vi "Set Setpoints.vi"(8 "error in":errorcluster, 10 "Plant Setpoints":T1, 11 "Sim Plant in":refnum<class "Sim Plant.lvclass">) -> (0 "error out":errorcluster, 3 "Sim Plant out":refnum<class "Sim Plant.lvclass">)   [LabVIEW 2026, in "Sim Plant.lvclass"]
doc: "Stores new plant setpoints. The plant model moves towards them on every Tick. Message: Set Setpoints Msg (payload Plant Setpoints)."
uses:
  Sim Plant.lvclass
  Sim Plant.lvclass/Sim Plant.ctl
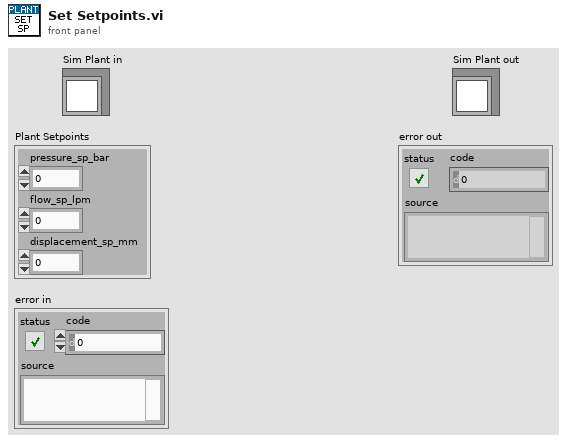
[diagram p1: front panel]
types:
  T1 = cluster{"pressure_sp_bar":dbl, "flow_sp_lpm":dbl, "displacement_sp_mm":dbl}
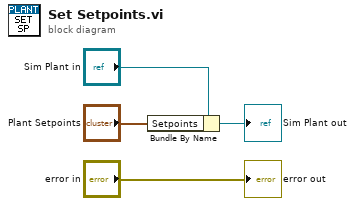
[diagram p0: block diagram]
diagram:
  n1 = Bundle By Name(cluster="Sim Plant in", "Setpoints"="Plant Setpoints") -> (→"Sim Plant out":refnum<class "Sim Plant.lvclass">)
  "error out" <- "error in"
